vi "Lire config Reg.vi"(2 "error in (no error)":errorcluster caption="entrée d'erreur (pas d'erreur)", 3 "refnum":T1) -> (0 "error out":errorcluster, 1 "refnum out":T1)   [LabVIEW 2022 SP3]
uses:
  <vilib>/Utility/config.llb/Config Data RefNum.ctl
  <vilib>/Utility/config.llb/Read Key (String).vi
  Variables globales/Variables glob EUROTHERM.vi
  <vilib>/Utility/config.llb/NI_LVConfig.lvlib
panel:
  out "Select regs acqui":cluster{"Sélect acqui 1COM reg":bool[]}[](array[cluster])
  out "Adresses regs dispo":cluster{"Adresses 1COM reg":dbl[]}[](array[cluster])
  out "Noms voies regs dispo":cluster{"Noms voies dispo 1COM":string[]}[](array[cluster])
  out "Ports COM REG":refnum<visa-resource-name>[](array[refnum])
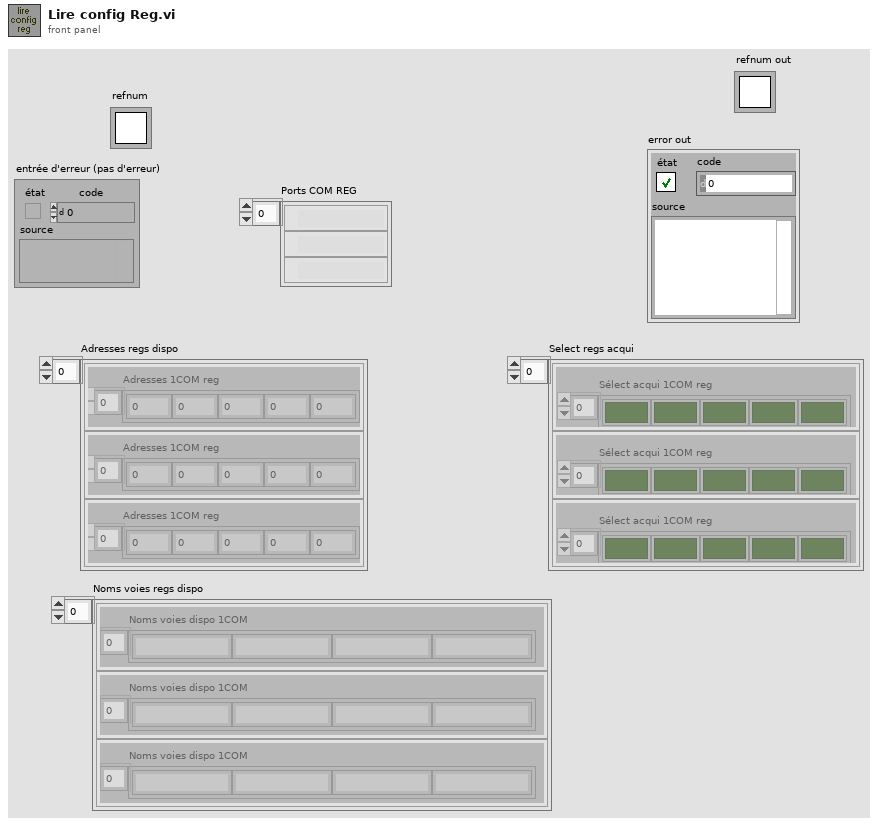
[diagram p1: front panel]
types:
  T1 = typedef "NI_LVConfig.lvlib/Config Data RefNum.ctl" = refnum<k1>
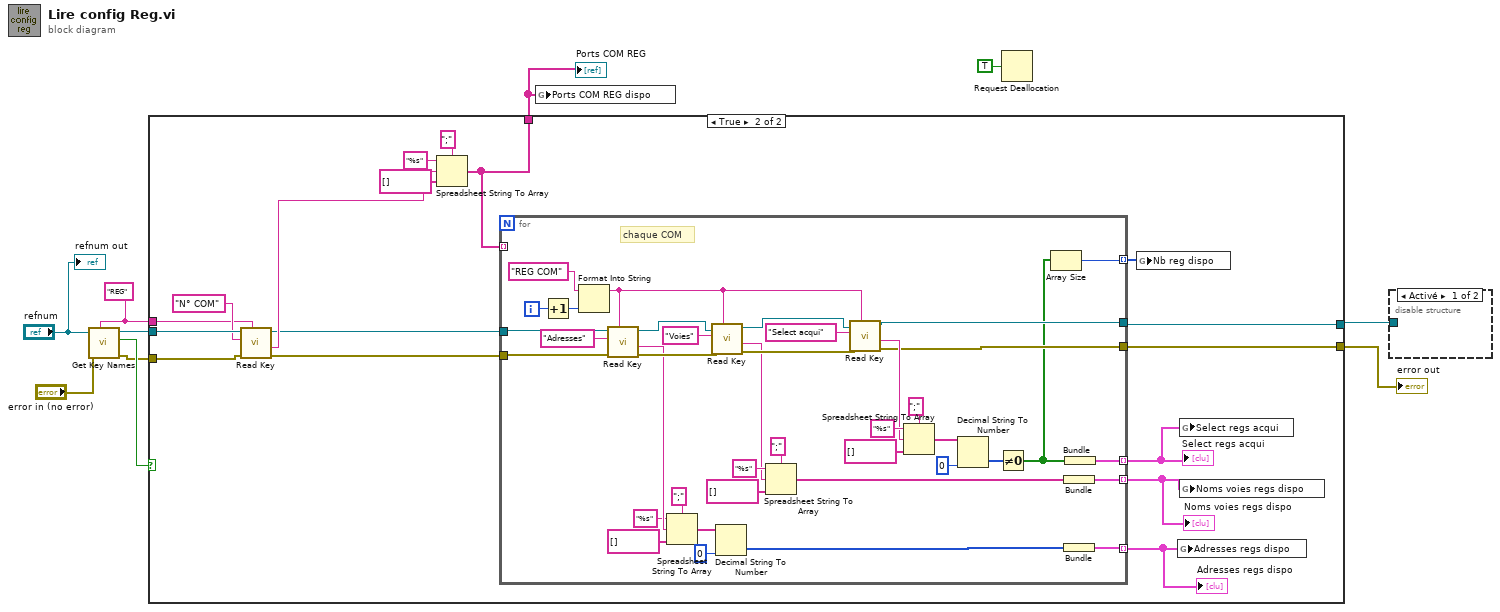
[diagram p0: block diagram]
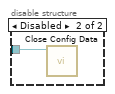
[diagram p2: hidden frame]
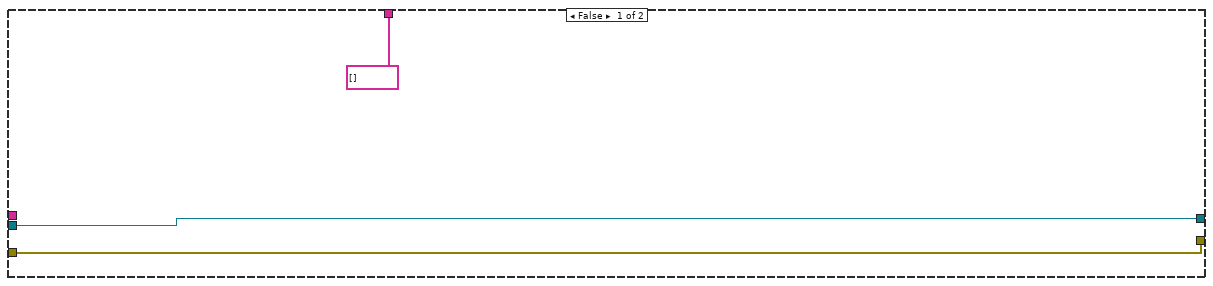
[diagram p3: hidden frame]
diagram:
  w6 = "REG" ("section")
  n1 = call <vilib>:"Get Key Names.vi"("section"=w6, "error in (no error)"="error in (no error)", "refnum"="refnum") -> ("error out"=w5:errorcluster, "section exists?"=w9:bool, "refnum out"=w4:T1)  [unwired: 5 in, 1 out]
  n2 = case shown="True" w9 {
    tunnel: w4 -> [w11 w30]
    tunnel: w5 -> [w13 w29]
    tunnel: w6 -> [_ w16]
    tunnel: [w13 w21] -> w7
    tunnel: [string[] [] ("type de tableau (2D de dbl)") w23] -> w1
    tunnel: [w11 w22] -> w2
    frame False {
    }
    frame True {
      n3 = call-poly <vilib>:"Read Key.vi"("section"=w16, "error in (no error)"=w29, "key"="N° COM", "refnum"=w30) -> ("error out"=w14:errorcluster, "value"=w25:string, "refnum out"=w15:T1)  [unwired: 4 in, 1 out]
      n4 = Spreadsheet String To Array(delimiter (Tab)=";" ("séparateur (Tabulation)"), format string="%s" ("chaîne de format"), spreadsheet string=w25, array type (2D Dbl)=string[] [] ("type de tableau (2D de dbl)")) -> (array=w23:string[])
      n5 = for {
        tunnel: w15 -> [w67]
        tunnel: w14 -> [w66]
        tunnel: w23 -> [_] mode=indexing
        tunnel: [w33] -> w22
        tunnel: [w32] -> w21
        tunnel: [w37] -> w17 mode=indexing
        tunnel: [w35] -> w19 mode=indexing
        tunnel: [w34] -> w18 mode=indexing
        tunnel: [w39] -> w20 mode=indexing
        i -> [w68]
        # "chaque COM"
        n6 = Increment(x=w68) -> (x+1=w47:i32)
        n7 = Format Into String(initial string="REG COM" ("chaîne"), w47) -> (resulting string=w58:string)  [unwired: 2 in, 1 out]
        n8 = call-poly <vilib>:"Read Key.vi"("section"=w58, "error in (no error)"=w66, "key"="Adresses", "refnum"=w67) -> ("error out"=w60:errorcluster, "value"=w57:string, "refnum out"=w62:T1)  [unwired: 4 in, 1 out]
        n9 = Spreadsheet String To Array(delimiter (Tab)=";" ("séparateur (Tabulation)"), format string="%s" ("chaîne de format"), spreadsheet string=w57, array type (2D Dbl)=string[] [] ("type de tableau (2D de dbl)")) -> (array=w53:string[])
        n10 = call-poly <vilib>:"Read Key.vi"("section"=w58, "error in (no error)"=w60, "key"="Voies", "refnum"=w62) -> ("error out"=w59:errorcluster, "value"=w49:string, "refnum out"=w61:T1)  [unwired: 4 in, 1 out]
        n11 = Decimal String To Number(string=w53, default (0L)=u8 0 ("valeur par défaut (0 I32)")) -> (number=w38:u8[])  [unwired: 1 in, 1 out]
        n12 = Spreadsheet String To Array(delimiter (Tab)=";" ("séparateur (Tabulation)"), format string="%s" ("chaîne de format"), spreadsheet string=w49, array type (2D Dbl)=string[] [] ("type de tableau (2D de dbl)")) -> (array=w36:string[])
        n13 = call-poly <vilib>:"Read Key.vi"("section"=w58, "error in (no error)"=w59, "key"="Select acqui", "refnum"=w61) -> ("error out"=w32:errorcluster, "value"=w43:string, "refnum out"=w33:T1)  [unwired: 4 in, 1 out]
        n14 = Spreadsheet String To Array(delimiter (Tab)=";" ("séparateur (Tabulation)"), format string="%s" ("chaîne de format"), spreadsheet string=w43, array type (2D Dbl)=string[] [] ("type de tableau (2D de dbl)")) -> (array=w41:string[])
        n15 = Decimal String To Number(string=w41, default (0L)=u8 0 ("valeur par défaut (0 I32)")) -> (number=w40:u8[])  [unwired: 1 in, 1 out]
        n16 = Not Equal To 0?(x=w40) -> (x != 0?=w31:bool[])
        n17 = Array Size(array=w31) -> (size(s)=w39:i32)
        n18 = Bundle("type de tableau (2D de dbl)"=w36) -> (w35:cluster{"type de tableau (2D de dbl)":string[]})  [unwired: 1 in]
        n19 = Bundle(w38) -> (w37:cluster{u8[]})  [unwired: 1 in]
        n20 = Bundle(w31) -> (w34:cluster{bool[]})  [unwired: 1 in]
      }
      "Noms voies regs dispo" <- w19
      "Adresses regs dispo" <- w17
      "Select regs acqui" <- w18
      n21 = global write "Variables glob EUROTHERM.vi" "Nb reg dispo"(w20) -> ()
      n22 = global write "Variables glob EUROTHERM.vi" "Adresses regs dispo"(w17) -> ()
      n23 = global write "Variables glob EUROTHERM.vi" "Select regs acqui"(w18) -> ()
      n24 = global write "Variables glob EUROTHERM.vi" "Noms voies regs dispo"(w19) -> ()
    }
  }
  "error out" <- w7
  "Ports COM REG" <- w1
  n25 = global write "Variables glob EUROTHERM.vi" "Ports COM REG dispo"(w1) -> ()
  n26 = Request Deallocation(TRUE ("flag")) -> ()
  n27 = disable-structure shown="Activé" {
    disable-tunnel: w2 -> [_ w70]
    frame Enabled {
    }
    frame Disabled {
      n28 = call <vilib>:"Close Config Data.vi"("refnum"=w70) -> ()  [unwired: 9 in, 2 out]
    }
  }
  "refnum out" <- "refnum"
